vi "Create.vi"(8 "error in (no error)":errorcluster) -> (0 "error out":errorcluster, 3 "Server out":refnum<class "Server.lvclass">)   [LabVIEW 2020, in "PV Access.lvlib" / "PVA Server.lvlib" / "Server.lvclass"]
doc: "Create a new server."
uses:
  Server.lvclass
  Source/Source.lvclass
  Server.lvclass/Server.ctl
  PV Access.lvlib
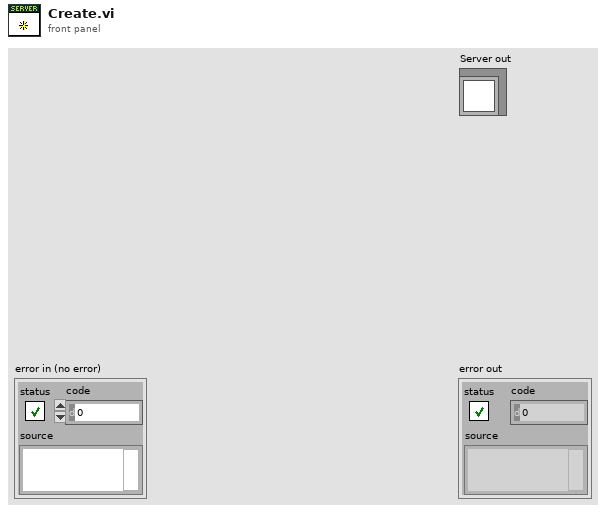
[diagram p1: front panel]
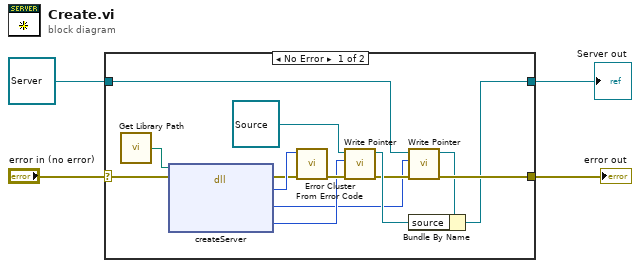
[diagram p0: block diagram]
diagram:
  n1 = case shown="No Error" "error in (no error)" {
    selector: "error in (no error)" -> [w18 w20]
    tunnel: [w8 w20] -> w2
    tunnel: [w6 w19] -> w3
    tunnel: refnum<class "Server.lvclass"> refnum ("Server in") -> [w9 w19]
    frame No Error {
      n2 = call "Get Library Path.vi"() -> ("Path"=w15:path)  [unwired: 1 in]
      n3 = dll-call lib="?" fn="createServer"(path in=w15, error in=w18) -> (error out=w16:errorcluster, "ret code"=w17:i32, "server"=w5:i64, "source"=w13:i64)  [unwired: 3 in, 1 out]
      n4 = call <vilib>:"Error Cluster From Error Code.vi"("error in (no error)"=w16, "error code (0)"=w17) -> ("error out"=w14:errorcluster)  [unwired: 7 in]
      n5 = call-dynamic "Write Pointer.vi"("error in (no error)"=w14, "Pointer"=w13, "Pointer Base in"=refnum<class "Source.lvclass"> refnum ("Source in")) -> ("error out"=w10:errorcluster, "Pointer Base out"=w11:refnum<class "Source.lvclass">)  [unwired: 7 in]
      n6 = call-dynamic "Write Pointer.vi"("error in (no error)"=w10, "Pointer"=w5, "Pointer Base in"=w9) -> ("error out"=w8:errorcluster, "Pointer Base out"=w7:refnum<class "Server.lvclass">)  [unwired: 7 in]
      n7 = Bundle By Name(cluster=w7, "source"=w11) -> (w6:refnum<class "Server.lvclass">)
    }
    frame Error {
    }
  }
  "error out" <- w2
  "Server out" <- w3
